vi "Center Object.vi"(8 "error in":errorcluster, 9 "Rectangle":T1, 10 "Scrollbar Visible?":bool, 11 "Dialog in":refnum<class "Dialog.lvclass">) -> (0 "error out":errorcluster, 3 "Dialog.lvclass out":refnum<class "Dialog.lvclass">)   [LabVIEW 2012, in "Dialog.lvlib" / "Dialog.lvclass"]
uses:
  Dialog.lvclass
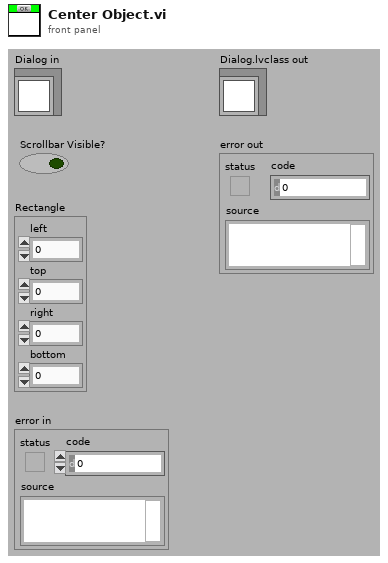
[diagram p1: front panel]
types:
  T1 = cluster{"left":i16, "top":i16, "right":i16, "bottom":i16}
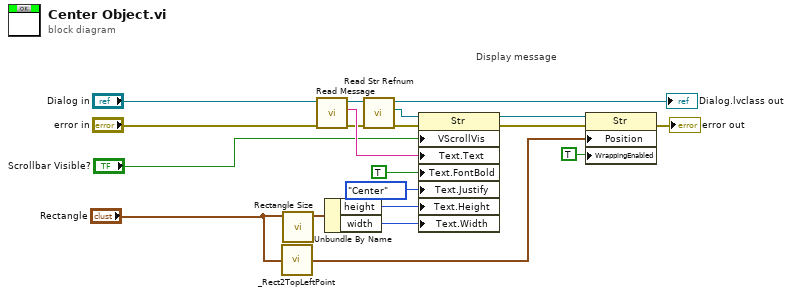
[diagram p0: block diagram]
diagram:
  # "Display message"
  n1 = call "_Rect2TopLeftPoint.vi"("bounds"="Rectangle") -> ("TopLeft point"=w4:cluster{"x":i32, "y":i32})  [unwired: 4 out]
  n2 = call "Rectangle Size.vi"("Rectangle"="Rectangle") -> ("Rect Size"=w20:cluster{"width":i32, "height":i32})  [unwired: 10 out]
  n3 = call-dynamic "Read Message.vi"("error in (no error)"="error in", "Dialog in"="Dialog in") -> ("error out"=w11:errorcluster, "Message"=w15:string, "Dialog out"=w12:refnum<class "Dialog.lvclass">)  [unwired: 7 out]
  n4 = Unbundle By Name(w20) -> ("height"=w17:i32, "width"=w18:i32)
  n5 = call-dynamic "Read Str Refnum.vi"("error in (no error)"=w11, "Dialog.lvclass in"=w12) -> ("error out"=w16:errorcluster, "Str Refnum"=w10:refnum<vi>, "Dialog.lvclass out"=→"Dialog.lvclass out":refnum<class "Dialog.lvclass">)  [unwired: 7 out]
  n6 = property class="Str"(reference=w10, error in=w16, "VScrollVis"="Scrollbar Visible?", "Text.Text"=w15, "Text.FontBold"=TRUE ("Size to Text?"), "Text.Justify"=enum16{"Left", "Center", "Right"}."Center" ("Justification"), "Text.Height"=w17, "Text.Width"=w18) -> (reference out=w3:refnum<vi>, error out=w2:errorcluster)
  n7 = property class="Str"(reference=w3, error in=w2, "Position"=w4, "WrappingEnabled"=TRUE ("Enable Wrapping")) -> (error out=→"error out":errorcluster)  [unwired: 1 out]
